vi "[ce] Find All Zeroes and Extrema of f(x).vi"(5 "accuracy":dbl=1e-08 format="%.2e", 6 "parameters":cluster{"name":string, "value":dbl}[](array[cluster]) {"value" format="%.2f"}, 7 "# points":u32=1000, 8 "error in":errorcluster, 9 "formula info":cluster{"formula":string, "x-variable":string}={"formula"="", "x-variable"="t"}, 10 "end":dbl=1.0 format="%.2f", 11 "start":dbl format="%.2f") -> (0 "error out":errorcluster, 1 "minima":cluster{"x":dbl[], "f(x)":dbl[]} {"f(x)" format="%.2f"; "x" format="%.2f"}, 2 "maxima":cluster{"x":dbl[], "f(x)":dbl[]} {"f(x)" format="%.2f"; "x" format="%.2f"}, 3 "zeroes":cluster{"x":dbl[], "f(x)":dbl[]} {"f(x)" format="%.2f"; "x" format="%.2f"}, 4 "ticks":u32)   [LabVIEW 2021]
doc: "The VI searches for all zeroes and local extrema of a 1D function in the specified interval. In addition, the VI allows specifying additional parameters and evaluating them in formula.\n\n::: CalcExpress Toolkit :::\nCopyright (c) 2000-2026 Konstantin Shifershteyn. All rights reserved."
panel:
  # "Example:\n\n accuracy: 1E-8 \n start: 0.0\n end: 1.0\n formula: x*x+sin(x)-1\n x-variable: x"
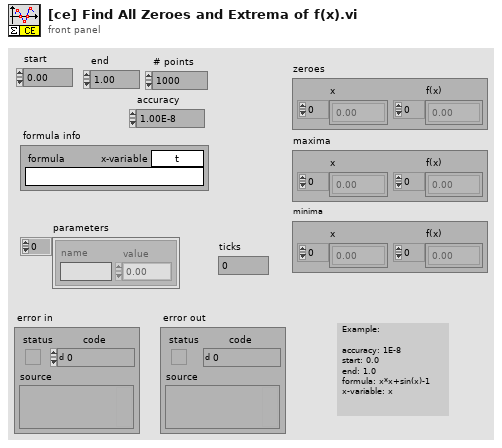
[diagram p1: front panel]
types:
  T1 = enum16{"create", "destroy", "set value", "get value"}
  T2 = typedef "VarMan Variable Context Handle.ctl" = i32
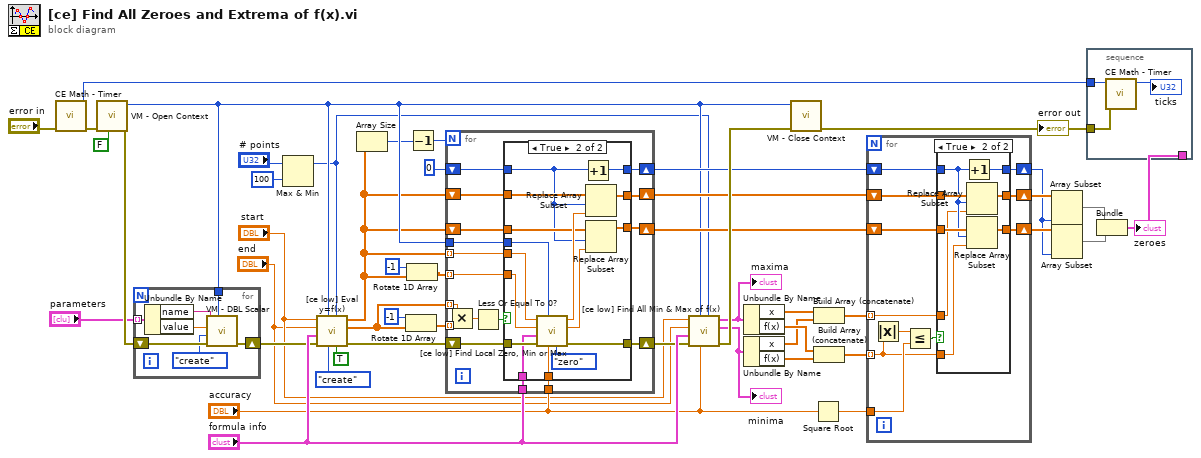
[diagram p0: block diagram]
diagram:
  n1 = call "CE Math - Timer.vi"("error in (no error)"="error in") -> ("error out"=w28:errorcluster, "ticks out"=w26:u32)  [unwired: 7 in]
  n2 = call "VM - Open Context.vi"("close loose contexts (F)"=FALSE ("close loose contexts (T)"), "error in"=w28) -> ("error out"=w19:errorcluster, "VC Handle out"=w20:T2)  [unwired: 7 in, 1 out]
  n3 = for {
    shift-right: [w52] -> w21
    shift-left: w19 -> [w53]
    tunnel: "parameters" -> [w50] mode=indexing
    tunnel: w20 -> [w49]
    n4 = Unbundle By Name(w50) -> ("name"=w54:string, "value"=w55:dbl)
    n5 = call "VM - DBL Scalar.vi"("VC Handle"=w49, "error in"=w53, "cmd"=T1."create", "value in"=w55, "name_spec"=w54) -> ("error out"=w52:errorcluster)  [unwired: 1 in, 5 out]
  }
  n6 = Max & Min(x="# points", y=u32 100) -> (max(x,y)=w6:u32)  [unwired: 1 out]
  n7 = call "[ce low] Eval y=f(x).vi"("include end point"=TRUE, "# points"=w6, "vm cmd"=T1."create", "VC Handle"=w20, "error in"=w21, "formula info"="formula info", "end"="end", "start"="start") -> ("error out"=w35:errorcluster, "f(x)"=w34:dbl[], "x"=w10:dbl[])  [unwired: 1 out]
  n8 = Array Size(array=w10) -> (size(s)=w9:i32)
  n9 = Rotate 1D Array(1:w34, 2:-1) -> (0:w47:dbl[])
  n10 = Rotate 1D Array(1:w10, 2:-1) -> (0:w45:dbl[])
  n11 = Decrement(x=w9) -> (x-1=w44:i32)
  n12 = for {
    N: w44 -> [_]
    tunnel: w34 -> [w72] mode=indexing
    tunnel: w47 -> [w71] mode=indexing
    shift-right: [w67] -> w23
    shift-left: w10 -> [w68]
    shift-right: [w65] -> w22
    shift-left: w10 -> [w66]
    tunnel: w10 -> [w64] mode=indexing
    tunnel: w45 -> [w63] mode=indexing
    shift-right: [w61] -> w32
    shift-left: w35 -> [w62]
    tunnel: w20 -> [w60]
    tunnel: "accuracy" -> [w59]
    tunnel: "formula info" -> [w58]
    shift-right: [w56] -> w24
    shift-left: 0 -> [w57]
    n13 = Multiply(x=w72, y=w71) -> (x*y=w70:dbl)
    n14 = Less Or Equal To 0?(x=w70) -> (x <= 0?=w69:bool)
    n15 = case shown="True" w69 {
      tunnel: w68 -> [w76 w81]
      tunnel: [w76 w79] -> w67
      tunnel: w66 -> [w75 w82]
      tunnel: [w75 w80] -> w65
      tunnel: w64 -> [_ w91]
      tunnel: w63 -> [_ w90]
      tunnel: w62 -> [w74 w92]
      tunnel: [w74 w89] -> w61
      tunnel: w60 -> [_ w88]
      tunnel: w59 -> [_ w87]
      tunnel: w58 -> [_ w86]
      tunnel: w57 -> [w73 w78]
      tunnel: [w73 w85] -> w56
      frame False {
      }
      frame True {
        n16 = call "[ce low] Find Local Zero, Min or Max.vi"("find"=enum16{"zero", "min", "max"}."zero", "accuracy"=w87, "VC Handle"=w88, "error in"=w92, "formula info"=w86, "end"=w90, "start"=w91) -> ("error out"=w89:errorcluster, "f(x)"=w83:dbl, "x"=w84:dbl)  [unwired: 2 in]
        n17 = Increment(x=w78) -> (x+1=w85:i32)
        n18 = Replace Array Subset(array=w81, new element=w84, index=w78) -> (w79:dbl[])
        n19 = Replace Array Subset(array=w82, new element=w83, index=w78) -> (w80:dbl[])
      }
    }
  }
  n20 = call "[ce low] Find All Min & Max of f(x).vi"("# points"=w6, "accuracy"="accuracy", "VC Handle"=w20, "error in"=w32, "formula info"="formula info", "end"="end", "start"="start") -> ("error out"=w36:errorcluster, "minima"=w12:cluster{"x":dbl[], "f(x)":dbl[]}, "maxima"=w13:cluster{"x":dbl[], "f(x)":dbl[]})  [unwired: 2 in]
  "minima" <- w12
  "maxima" <- w13
  n21 = Unbundle By Name(w13) -> ("x"=w43:dbl[], "f(x)"=w42:dbl[])
  n22 = Unbundle By Name(w12) -> ("x"=w41:dbl[], "f(x)"=w40:dbl[])
  n23 = call "VM - Close Context.vi"("error in"=w36, "VC Handle"=w20) -> ("error out"=w31:errorcluster)  [unwired: 8 in, 1 out]
  "error out" <- w31
  n24 = Square Root(x="accuracy") -> (sqrt(x)=w11:dbl)
  n25 = Build Array (concatenate)(w43, w41) -> (w29:dbl[])
  n26 = Build Array (concatenate)(w42, w40) -> (w25:dbl[])
  n27 = for {
    shift-right: [w93] -> w38
    shift-left: w22 -> [w94]
    shift-right: [w95] -> w39
    shift-left: w23 -> [w96]
    tunnel: w29 -> [w97] mode=indexing
    tunnel: w25 -> [w98] mode=indexing
    shift-right: [w99] -> w37
    shift-left: w24 -> [w100]
    tunnel: w11 -> [w102]
    n28 = Absolute Value(x=w98) -> (abs(x)=w103:dbl)
    n29 = Less Or Equal?(x=w103, y=w102) -> (x <= y?=w101:bool)
    n30 = case shown="True" w101 {
      tunnel: w100 -> [w106 w109]
      tunnel: [w106 w112] -> w99
      tunnel: w98 -> [_ w107]
      tunnel: w97 -> [_ w108]
      tunnel: w96 -> [w105 w114]
      tunnel: [w105 w113] -> w95
      tunnel: w94 -> [w104 w111]
      tunnel: [w104 w110] -> w93
      frame False {
      }
      frame True {
        n31 = Increment(x=w109) -> (x+1=w112:i32)
        n32 = Replace Array Subset(array=w114, new element=w108, index=w109) -> (w113:dbl[])
        n33 = Replace Array Subset(array=w111, new element=w107, index=w109) -> (w110:dbl[])
      }
    }
  }
  n34 = Array Subset(array=w39, length=w37) -> (w16:dbl[])  [unwired: 1 in]
  n35 = Array Subset(array=w38, length=w37) -> (w15:dbl[])  [unwired: 1 in]
  n36 = Bundle(w16, w15) -> (w14:cluster{dbl[], dbl[]})  [unwired: 1 in]
  "zeroes" <- w14
  n37 = stacked-sequence {
    tunnel: w26 -> [w117]
    tunnel: w31 -> [w116]
    tunnel: w14 -> [_]
    frame #0 {
      n38 = call "CE Math - Timer.vi"("error in (no error)"=w116, "ticks in"=w117) -> ("ticks out"=→"ticks":u32)  [unwired: 6 in, 1 out]
    }
  }
